vi "Delete RPC Client Method Template Files.vi"(8 "error in (no error)":errorcluster, 11 "library in":refnum<vi>) -> (0 "error out":errorcluster, 3 "library out":refnum<vi>)   [LabVIEW 2019, in "gRPC Template Creation Utility.lvlib"]
uses:
  gRPC Template Creation Utility.lvlib
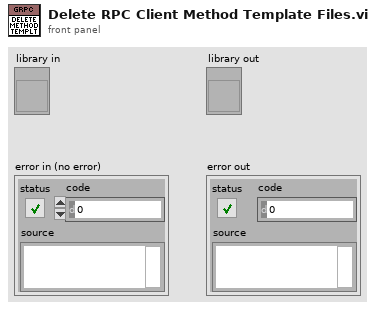
[diagram p1: front panel]
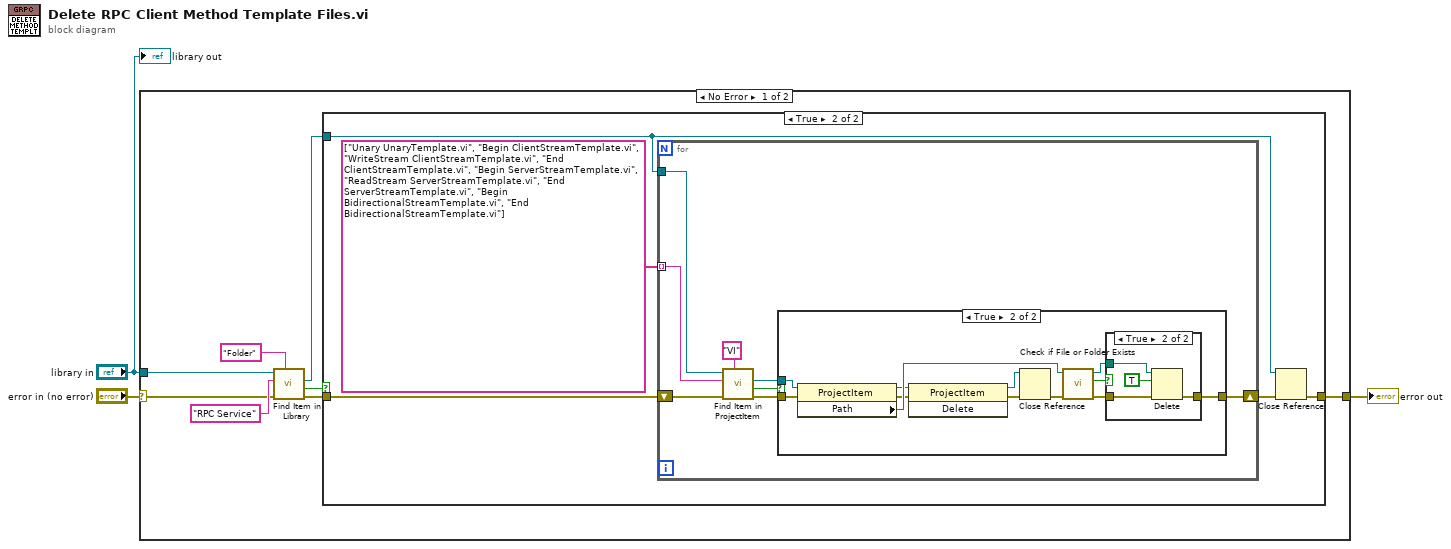
[diagram p0: block diagram]
diagram:
  n1 = case shown="No Error" "error in (no error)" {
    selector: "error in (no error)" -> [w5 w44]
    tunnel: "library in" -> [w9 _]
    tunnel: [w4 w44] -> w1
    frame No Error {
      n2 = call "Find Item in Library.vi"("Item Type"="Folder", "error in (no error)"=w5, "Item Name"="RPC Service", "Library item in"=w9) -> ("error out"=w7:errorcluster, "Found?"=w6:bool, "Project Item (Library Item)"=w8:refnum<vi>)  [unwired: 4 in, 1 out]
      n3 = case shown="True" w6 {
        tunnel: w8 -> [_ w15]
        tunnel: w7 -> [w12 w17]
        tunnel: [w12 w13] -> w4
        frame False {
        }
        frame True {
          n4 = for {
            tunnel: w15 -> [w25]
            shift-right: [w19] -> w14
            shift-left: w17 -> [w21]
            tunnel: string[] ["Unary UnaryTemplate.vi", "Begin ClientStreamTemplate.vi", "WriteStream ClientStreamTemplate.vi", "End ClientStreamTemplate.vi", "Begin ServerStreamTemplate.vi", "ReadStream ServerStreamTemplate.vi", "End ServerStreamTemplate.vi", "Begin BidirectionalStreamTemplate.vi", "End BidirectionalStreamTemplate.vi"] -> [w18] mode=indexing
            n5 = call "Find Item in ProjectItem.vi"("Item Type"="VI", "error in (no error)"=w21, "Name"=w18, "ProjectItem in"=w25) -> ("error out"=w20:errorcluster, "Found ?"=w23:bool, "Item Refnum out"=w22:refnum<vi>)  [unwired: 4 in, 1 out]
            n6 = case shown="True" w23 {
              tunnel: w20 -> [w26 w38]
              tunnel: w22 -> [_ w37]
              tunnel: [w26 w32] -> w19
              frame False {
              }
              frame True {
                n7 = property class="ProjectItem"(reference=w37, error in=w38) -> (reference out=w29:refnum<vi>, error out=w30:errorcluster, "Path"=w33:path)
                n8 = invoke class="ProjectItem" method="Delete"(reference=w29, error in=w30) -> (reference out=w31:refnum<vi>, error out=w27:errorcluster)  [unwired: 1 in, 1 out]
                n9 = Close Reference(reference=w31, error in (no error)=w27) -> (error out=w28:errorcluster)
                n10 = call <vilib>:"Check if File or Folder Exists.vi"("error in (no error)"=w28, "path"=w33) -> ("error out"=w36:errorcluster, "file or folder exists?"=w34:bool, "dup path"=w35:path)  [unwired: 7 in]
                n11 = case shown="True" w34 {
                  tunnel: w35 -> [_ w43]
                  tunnel: w36 -> [w39 w42]
                  tunnel: [w39 w41] -> w32
                  frame False {
                  }
                  frame True {
                    n12 = Delete(path (use dialog)=w43, entire hierarchy (F)=TRUE, error in=w42) -> (error out=w41:errorcluster)  [unwired: 2 in, 2 out]
                  }
                }
              }
            }
          }
          n13 = Close Reference(reference=w15, error in (no error)=w14) -> (error out=w13:errorcluster)
        }
      }
    }
    frame Error {
    }
  }
  "error out" <- w1
  "library out" <- "library in"
